vi "CommonVIs_UpdateAttributeCtrlPath.vi"(10 "ClassInfo":T1[](array[typedef]), 11 "DataType in":T2) -> (3 "DataType out":T2)   [LabVIEW 2020]
uses:
  CommonVIs_AttributeType.ctl
  CommonVIs_AttributeDataType.ctl
  String/GDSString_AccessScopeModifierType.ctl
  CommonVIs_ClassNamePathType.ctl
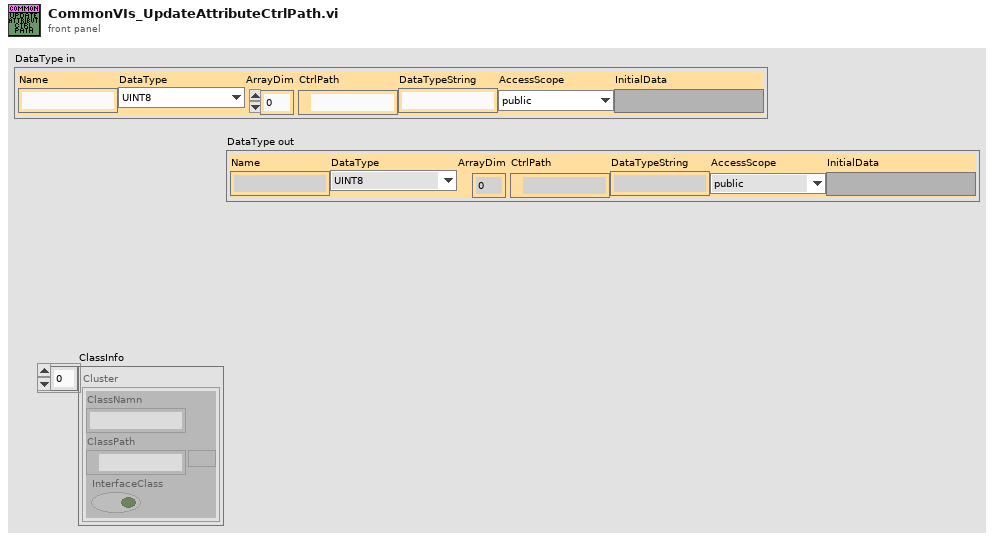
[diagram p1: front panel]
types:
  T1 = typedef "CommonVIs_ClassNamePathType.ctl" = cluster{"ClassNamn":string, "ClassPath":path, "InterfaceClass":bool}
  T2 = typedef "CommonVIs_AttributeType.ctl" = cluster{"Name":string, "DataType":T3, "ArrayDim":i32, "CtrlPath":path, "DataTypeString":string, "AccessScope":T4, "InitialData":variant}
  T3 = typedef "CommonVIs_AttributeDataType.ctl" = enum16{"UINT8", "INT8", "UINT16", "INT16", "UINT32", "INT32", "UINT64", "INT64", "SGL", "DBL", "EXT", "CSG", "CDB", "CXT", "TimeStamp", "STRING", "PATH", "BOOL", "ENUM", "RefNum", "VIRefNum", "LabVIEW Class", "Cluster", "Variant", "TypeDef", "Waveform", "LabVIEW Object", "Other", "void", "Set", "Map"}
  T4 = typedef "GDSString_AccessScopeModifierType.ctl" = enum16{"public", "private", "protected", "internal"}
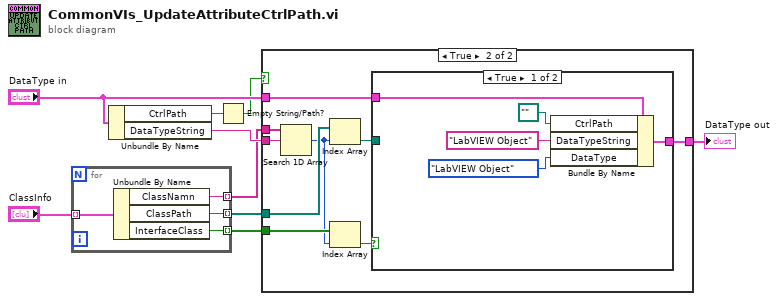
[diagram p0: block diagram]
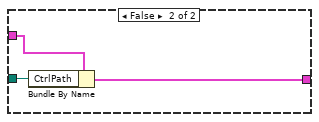
[diagram p3: hidden frame]
diagram:
  n1 = for {
    tunnel: "ClassInfo" -> [w13] mode=indexing
    tunnel: [w12] -> w3 mode=indexing
    tunnel: [w11] -> w2 mode=indexing
    tunnel: [w10] -> w1 mode=indexing
    n2 = Unbundle By Name(w13) -> ("ClassNamn"=w12:string, "ClassPath"=w11:path, "InterfaceClass"=w10:bool)
  }
  n3 = Unbundle By Name("DataType in") -> ("CtrlPath"=w5:path, "DataTypeString"=w7:string)
  n4 = Empty String/Path?(string/path=w5) -> (empty?=w6:bool)
  n5 = case shown="True" w6 {
    tunnel: w7 -> [_ w23]
    tunnel: w3 -> [_ w22]
    tunnel: w2 -> [_ w21]
    tunnel: "DataType in" -> [w14 w20]
    tunnel: [w14 w19] -> w9
    tunnel: w1 -> [_ w17]
    frame False {
    }
    frame True {
      n6 = Search 1D Array(1D array=w22, element=w23) -> (index of element=w16:i32)  [unwired: 1 in]
      n7 = Index Array(array=w21, index=w16) -> (element=w18:path)
      n8 = Index Array(array=w17, index=w16) -> (element=w15:bool)
      n9 = case shown="True" w15 {
        tunnel: w20 -> [w28 w31]
        tunnel: [w27 w30] -> w19
        tunnel: w18 -> [_ w29]
        frame True {
          n10 = Bundle By Name(cluster=w28, "CtrlPath"=path "", "DataTypeString"="LabVIEW Object", "DataType"=CommonVIs_AttributeDataType."LabVIEW Object") -> (w27:T2)
        }
        frame False {
          n11 = Bundle By Name(cluster=w31, "CtrlPath"=w29) -> (w30:T2)
        }
      }
    }
  }
  "DataType out" <- w9
